vi "Async Spawn Child.vi"(4 "UID":string, 7 "Actor in":refnum<class "Actor.lvclass">, 9 "Mid Actors":refnum<class "Actor.lvclass">[](array[class])) -> (0 "Error out":errorcluster, 5 "Actor out":refnum<class "Actor.lvclass">)   [LabVIEW 2020, in "jettl.lvlib"]
uses:
  jettl.lvlib
  Actor/Actor.lvclass
  Transport/Transport.lvclass
  Attributes.ctl
  Attributes/Attributes.lvclass
  Msgs.ctl
  Msg/Msg.lvclass
  Base Attributes/Base Attributes/Base Attributes.lvclass/Base Attributes.ctl
  Unify Iterator.vi
  Find Child UIDs.vi
  Base Attributes/Base Attributes/Base Attributes.lvclass
  C:/git/jettl/src/jettl/jettl/Attributes/Attributes.lvclass
  Already In Stop--error.vi
  Not Concrete Actor--error.vi
  UID Empty--error.vi
  UID Already Exists--error.vi
  Base Attributes/Base Attributes.lvlib
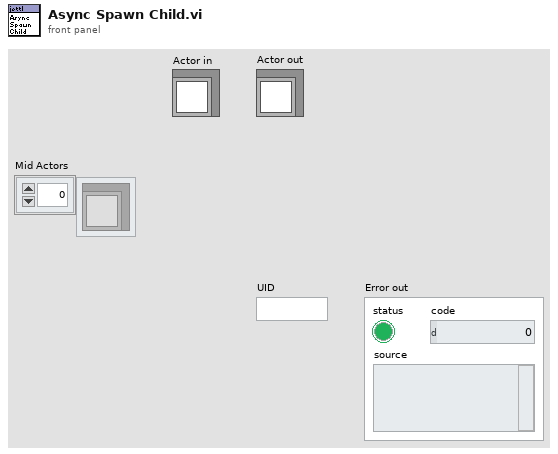
[diagram p1: front panel]
types:
  T1 = typedef "jettl.lvlib/Attributes.ctl" = cluster{"Unified Msgs":T2, "Edge Actors":refnum<class "Actor.lvclass">[], "Core Actors":refnum<class "Actor.lvclass">[], "Parent Attributes":refnum<class "Attributes.lvclass">, "Root":bool, "App Ref":refnum<vi>, "UID":string, "Transport":refnum<class "Transport.lvclass">, "VI Ref":refnum<vi>, "Actors":refnum<class "Actor.lvclass">[]}
  T2 = typedef "jettl.lvlib/Msgs.ctl" = set{refnum<class "Msg.lvclass">}
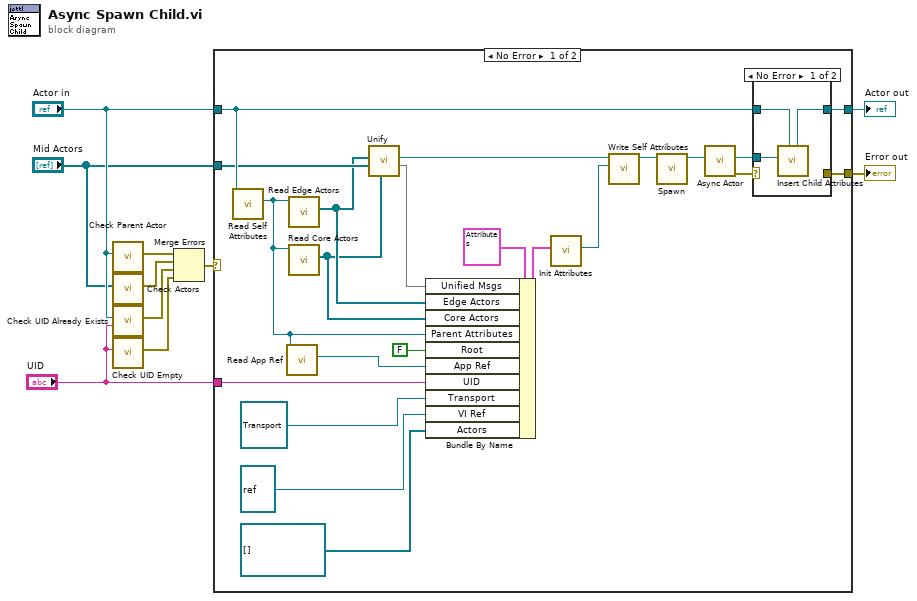
[diagram p0: block diagram]
diagram:
  n1 = call "Check Parent Actor.vi"("Actor"="Actor in") -> ("Error"=w8:errorcluster)  [unwired: 10 in]
  n2 = call "Check Actors.vi"("Actors"="Mid Actors") -> ("Error"=w1:errorcluster)  [unwired: 10 in]
  n3 = call "Check UID Already Exists.vi"("UID"="UID", "Actor"="Actor in") -> ("Error"=w6:errorcluster)  [unwired: 9 in]
  n4 = call "Check UID Empty.vi"("UID"="UID") -> ("Error"=w5:errorcluster)  [unwired: 10 in]
  n5 = Merge Errors(w8, w1, w6, w5) -> (w7:errorcluster)
  n6 = case shown="No Error" w7 {
    selector: w7 -> [_ w38]
    tunnel: "Actor in" -> [w29 w39]
    tunnel: [w32 w38] -> w10
    tunnel: [w31 w39] -> w9
    tunnel: "UID" -> [w24 _]
    tunnel: "Mid Actors" -> [w15 _]
    frame No Error {
      n7 = call-dynamic "Read Self Attributes.vi"("Actor in"=w29) -> ("Self Attributes"=w16:refnum<class "Attributes.lvclass">)  [unwired: 10 in]
      n8 = call-dynamic "Read App Ref.vi"("Attributes in"=w16) -> ("App Ref"=w17:refnum<vi>)  [unwired: 10 in]
      n9 = call-dynamic "Read Edge Actors.vi"("Attributes in"=w16) -> ("Edge Actors"=w14:refnum<class "Actor.lvclass">[])  [unwired: 10 in]
      n10 = call-dynamic "Read Core Actors.vi"("Attributes in"=w16) -> ("Core Actors"=w13:refnum<class "Actor.lvclass">[])  [unwired: 10 in]
      n11 = call "Unify.vi"("Core Actors"=w13, "Mid Actors"=w15, "Edge Actors"=w14) -> ("Unified Msgs"=w12:T2, "Unified Actor"=w11:refnum<class "Actor.lvclass">)  [unwired: 7 in]
      n12 = Bundle By Name(cluster=T1 {"Unified Msgs"={}, "Edge Actors"=[], "Core Actors"=[], "Parent Attributes"=refnum, "Root"=FALSE, "App Ref"=refnum, "UID"="", "Transport"=refnum, "VI Ref"=refnum, "Actors"=[]} ("Attributes"), "Unified Msgs"=w12, "Edge Actors"=w14, "Core Actors"=w13, "Parent Attributes"=w16, "Root"=FALSE, "App Ref"=w17, "UID"=w24, "Transport"=refnum<class "Transport.lvclass"> refnum, "VI Ref"=refnum<vi> refnum ("Actor Ref"), "Actors"=refnum<class "Actor.lvclass">[] []) -> (w22:T1)
      n13 = call "Init Attributes.vi"("Attributes"=w22) -> ("Attributes"=w30:refnum<class "Attributes.lvclass">)  [unwired: 10 in]
      n14 = call-dynamic "Write Self Attributes.vi"("Self Attributes"=w30, "Actor in"=w11) -> ("Actor out"=w21:refnum<class "Actor.lvclass">)  [unwired: 9 in]
      n15 = call-dynamic "Spawn.vi"("Actor in"=w21) -> ("Actor out"=w20:refnum<class "Actor.lvclass">)  [unwired: 10 in]
      n16 = call "Async Actor.vi"("Unified Actor"=w20) -> ("Error out"=w18:errorcluster, "Child Attributes"=w19:refnum<class "Attributes.lvclass">)  [unwired: 9 in]
      n17 = case shown="No Error" w18 {
        selector: w18 -> [_ w36]
        tunnel: w29 -> [w35 w37]
        tunnel: [w34 w37] -> w31
        tunnel: w19 -> [w33 _]
        tunnel: [_ w36] -> w32
        frame No Error {
          n18 = call "Insert Child Attributes.vi"("Actor in"=w35, "Child Attributes"=w33) -> ("Actor out"=w34:refnum<class "Actor.lvclass">)  [unwired: 9 in]
        }
        frame Error {
        }
      }
    }
    frame Error {
    }
  }
  "Actor out" <- w9
  "Error out" <- w10
